vi "LTE check RB Szie.vi"(8 "error in (no error)":errorcluster caption="에러 입력(에러 없음)", 11 "Instrument Manager 입력":refnum<class "Instrument Manager.lvclass">) -> (0 "error out":errorcluster caption="에러 출력", 2 "불리언":bool, 3 "Instrument Manager 출력":refnum<class "Instrument Manager.lvclass">)   [LabVIEW 2023, in "Instrument Manager.lvclass"]
uses:
  Instrument Manager.lvclass
  Module/ANRITSU Call Box/Type Definition/LTE RB Setting Params for query.ctl
  Instrument Manager.lvclass/Instrument Manager.ctl
  Module/ANRITSU Call Box/Interface Class/Anritsu Call Box.lvclass
  Module/ANRITSU Call Box/ANRITSU Call Box.lvlib
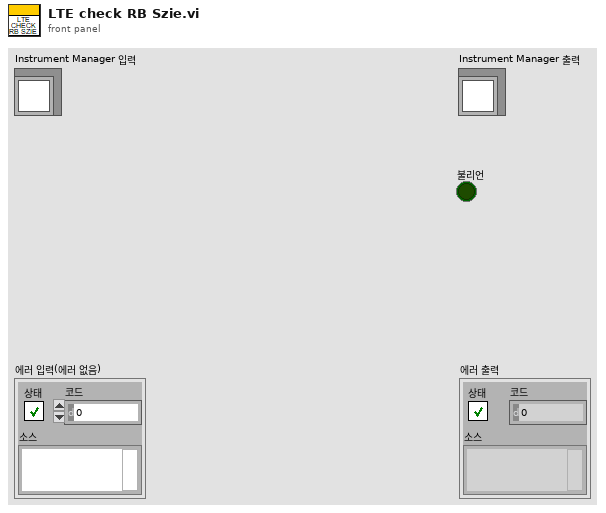
[diagram p1: front panel]
types:
  T1 = typedef "ANRITSU Call Box.lvlib/LTE RB Setting Params for query.ctl" = cluster{"Target CA Type":enum16{"PCC", "SCC1"}, "RB Setting Type":enum16{"Number of RB", "Starting RB"}}
  T2 = cluster{"Anritsu Call Box":refnum<class "Anritsu Call Box.lvclass">, "Spectrum Analyzer":refnum<class "Interface_Spectrum.lvclass">, "RF Switch Box":refnum<class "RF Filter Box.lvclass">, "Turn Table":refnum<class "Interface - Turn Table.lvclass">, "Mast":refnum<class "Interface - Mast.lvclass">, "3D Controller":refnum<class "Interface_3D Controller.lvclass">}
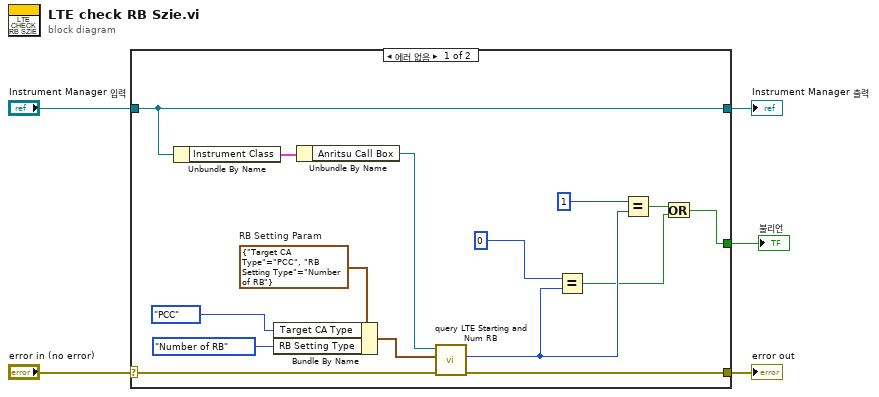
[diagram p0: block diagram]
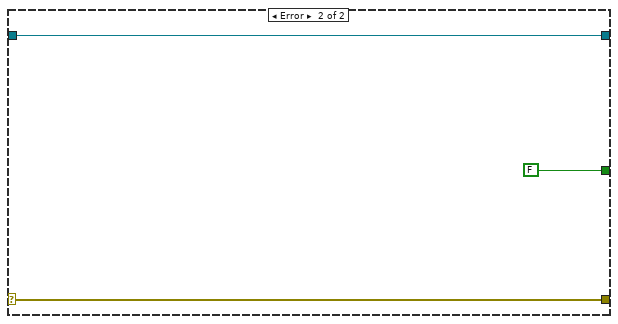
[diagram p2: hidden frame]
diagram:
  n1 = case shown="에러 없음" "error in (no error)" {
    selector: "error in (no error)" -> [w17 w23]
    tunnel: [w15 w23] -> w4
    tunnel: [w14 w22] -> w2
    tunnel: "Instrument Manager 입력" -> [w14 w22]
    tunnel: [w6 FALSE] -> w1
    frame No Error {
      w20 = T1 {"Target CA Type"=enum."PCC", "RB Setting Type"=enum."Number of RB"}  # RB Setting Param
      n2 = Unbundle By Name(w14) -> ("Instrument Class"=w13:T2)
      n3 = Bundle By Name(cluster=w20, "Target CA Type"=enum16{"PCC", "SCC1"}."PCC", "RB Setting Type"=enum16{"Number of RB", "Starting RB"}."Number of RB") -> (w16:T1)
      n4 = Unbundle By Name(w13) -> ("Anritsu Call Box"=w12:refnum<class "Anritsu Call Box.lvclass">)
      n5 = call-dynamic "query LTE Starting and Num RB.vi"("error in (no error)"=w17, "RB Setting Param"=w16, "Anritsu Call Box in"=w12) -> ("error out"=w15:errorcluster, "RB Value"=w9:i32)  [unwired: 6 in, 1 out]
      n6 = Equal?(x=0, y=w9) -> (x = y?=w7:bool)
      n7 = Equal?(x=1, y=w9) -> (x = y?=w8:bool)
      n8 = Or(x=w8, y=w7) -> (x .or. y?=w6:bool)
    }
    frame Error {
    }
  }
  "error out" <- w4
  "Instrument Manager 출력" <- w2
  "불리언" <- w1
